vi "Flow_Control.vi"() -> ()   [LabVIEW 2026]
panel:
  in  "reset_emergency":bool
  in  "stop_simulation":bool
  in  "emergency_stop":bool
  out "flow_rate_chart":dbl(graph)
  out "valve_open":bool
  out "flow_rate (L/min)":dbl
  in  "valve_opening (%)":dbl min=0.0 max=100.0 step=1.0
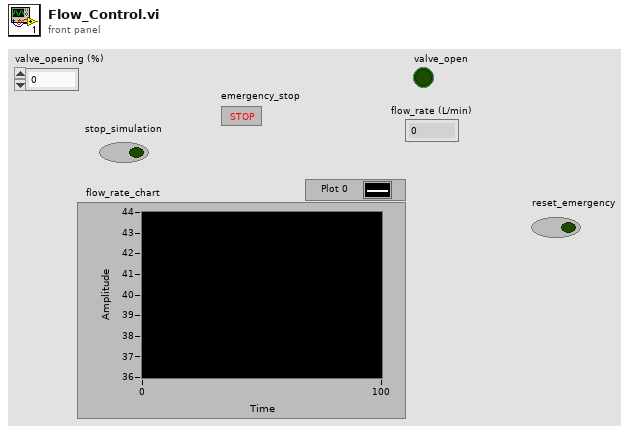
[diagram p1: front panel]
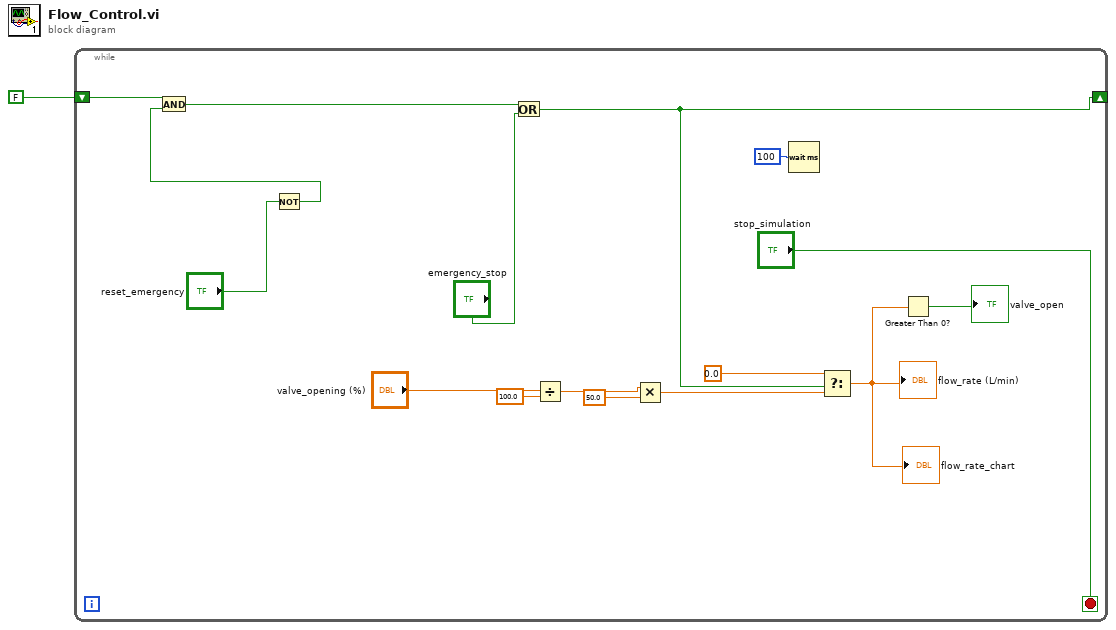
[diagram p0: block diagram]
diagram:
  n1 = while {
    shift-right: [w2] -> _
    shift-left: FALSE -> [w6]
    stop <- "stop_simulation" stop-if-true
    n2 = Not(x="reset_emergency") -> (.not. x?=w5:bool)
    n3 = And(x=w6, y=w5) -> (x .and. y?=w4:bool)
    n4 = Or(x=w4, y="emergency_stop") -> (x .or. y?=w2:bool)
    n5 = Divide(x="valve_opening (%)", y=100.0) -> (x/y=w15:dbl)
    n6 = Multiply(x=w15, y=50.0) -> (x*y=w13:dbl)
    n7 = Wait (ms)(milliseconds to wait=u32 100) -> ()  [unwired: 1 out]
    n8 = Select(t=0.0, s=w2, f=w13) -> (s? t:f=w11:dbl)
    "flow_rate (L/min)" <- w11
    "flow_rate_chart" <- w11
    n9 = Greater Than 0?(x=w11) -> (x > 0?=→"valve_open":bool)
  }
